vi "CANsub_WS_Close.vi"(7 "cert path":path=path "/home/lvuser/cansub_root_cert.crt", 8 "error in (no error)":errorcluster, 9 "channel":u8=2, 10 "host":string, 11 "TLS Connection":refnum<k5>) -> (0 "error out":errorcluster, 3 "closed by device":bool)   [LabVIEW 2021, in "CANsub_Common.lvlib"]
doc: "Closes the CANsub WebSocket: sends close frame 1000, reads until the device closes TCP (max 2 s), closes TCP. If the device did not close it, frees the channel with DELETE /api/can/<ch>/ws (200 or 404 OK). Always runs, also with an error in; the original error comes first in error out."
uses:
  CANsub_Common.lvlib
  <vilib>/httpClient/LabVIEWHTTPClient.lvlib
  Typedefs/HTTP_Method.ctl
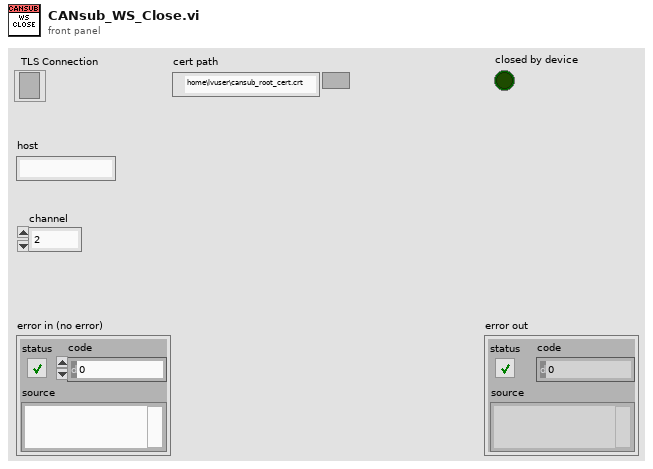
[diagram p1: front panel]
types:
  T1 = enum16{"Standard", "Buffered", "CRLF", "Immediate"}
  T2 = typedef "CANsub_Common.lvlib/HTTP_Method.ctl" = enum16{"GET", "PUT", "POST", "DELETE"}
  T3 = typedef "LabVIEWHTTPClient.lvlib/ClientHandle.ctl" = refnum<k1>
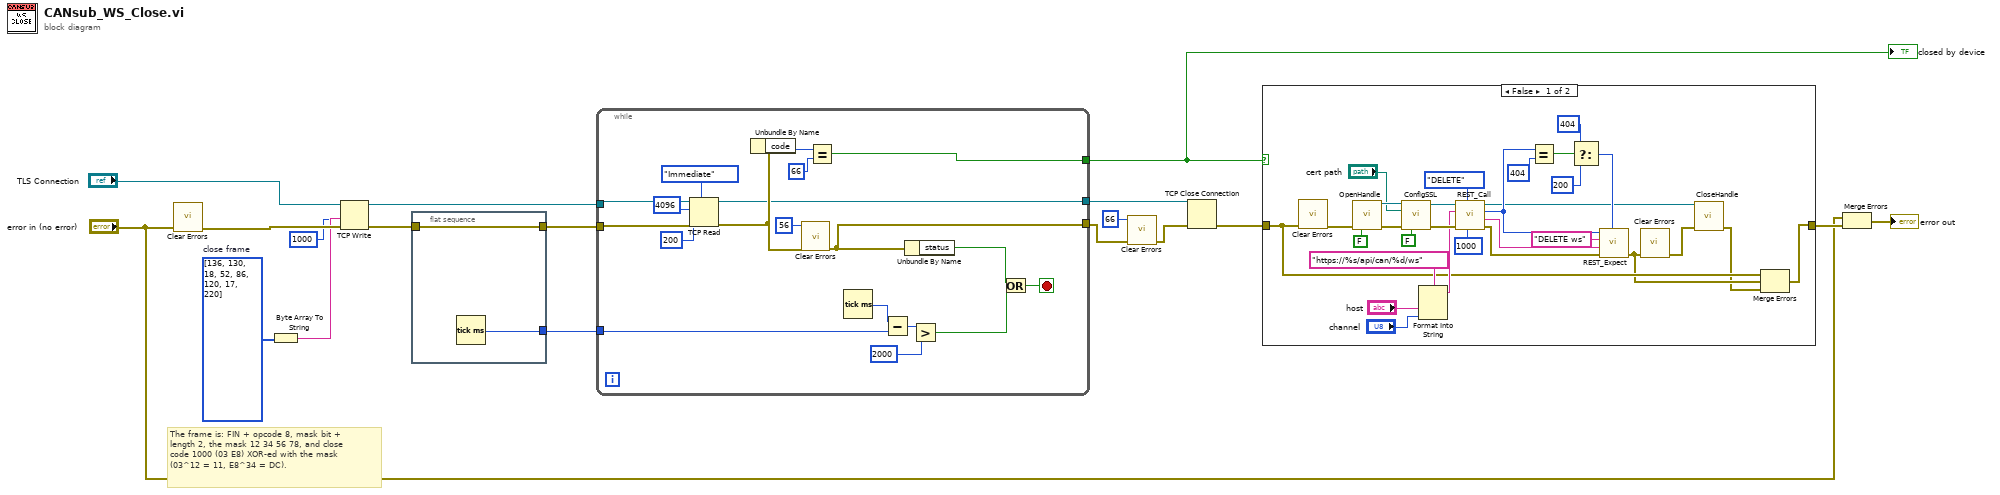
[diagram p0: block diagram]
diagram:
  w18 = u8[] [136, 130, 18, 52, 86, 120, 17, 220]  # close frame
  # "The frame is: FIN + opcode 8, mask bit + length 2, the mask 12 34 56 78, and close code 1000 (03 E8) XOR-ed with the mask (03^12 = 11, E8^34 = DC)."
  n1 = call <vilib>:"Clear Errors.vi"("error in (no error)"="error in (no error)") -> ("error out"=w17:errorcluster)  [unwired: 5 in, 1 out]
  n2 = Byte Array To String(unsigned byte array=w18) -> (string=w15:string)
  n3 = TCP Write(connection ID="TLS Connection", data in=w15, error in (no error)=w17, 9:1000 ("timeout ms (25000)")) -> (connection ID out=w7:refnum<k5>, error out=w13:errorcluster)  [unwired: 1 out]
  n4 = flat-sequence {
    tunnel: w13 -> [w20]
    tunnel: [w20] -> w11
    tunnel: [w19] -> w10
    frame #0 {
      n5 = Tick Count (ms)() -> (millisecond timer value=w19:u32)
    }
  }
  n6 = while {
    tunnel: w11 -> [w37]
    tunnel: w7 -> [w34]
    tunnel: w10 -> [w29]
    tunnel: [w23] -> w9
    tunnel: [w22] -> w2
    tunnel: [w21] -> w1
    stop <- w24 stop-if-true
    n7 = TCP Read(connection ID=w34, bytes to read=4096, error in (no error)=w37, 7:T1."Immediate" ("mode (standard)"), 9:200 ("timeout ms (25000)")) -> (connection ID out=w21:refnum<k5>, error out=w31:errorcluster)  [unwired: 1 out]
    n8 = Unbundle By Name(w31) -> ("code"=w33:i32)
    n9 = call <vilib>:"Clear Errors.vi"("error in (no error)"=w31, "specific error code to clear (0: all)"=56) -> ("error out"=w23:errorcluster)  [unwired: 4 in, 1 out]
    n10 = Equal?(x=w33, y=66) -> (x = y?=w22:bool)
    n11 = Tick Count (ms)() -> (millisecond timer value=w30:u32)
    n12 = Subtract(x=w30, y=w29) -> (x-y=w28:u32)
    n13 = Unbundle By Name(w23) -> ("status"=w26:bool)
    n14 = Greater?(x=w28, y=u32 2000) -> (0:w25:bool)
    n15 = Or(x=w26, y=w25) -> (x .or. y?=w24:bool)
  }
  "closed by device" <- w2
  n16 = call <vilib>:"Clear Errors.vi"("error in (no error)"=w9, "specific error code to clear (0: all)"=66) -> ("error out"=w8:errorcluster)  [unwired: 4 in, 1 out]
  n17 = TCP Close Connection(connection ID=w1, error in (no error)=w8) -> (error out=w6:errorcluster)  [unwired: 1 in, 1 out]
  n18 = case shown="False" w2 {
    tunnel: w6 -> [w44 w69]
    tunnel: [w41 w69] -> w5
    frame False {
      n19 = call <vilib>:"Clear Errors.vi"("error in (no error)"=w44) -> ("error out"=w68:errorcluster)  [unwired: 5 in, 1 out]
      n20 = call <vilib>:"OpenHandle.vi"("error in (no error)"=w68, "verify server(true)"=FALSE) -> ("client handle out"=w66:T3, "error out"=w65:errorcluster)  [unwired: 12 in]
      n21 = call <vilib>:"ConfigSSL.vi"("client handle"=w66, "CA certificate file"="cert path", "error in (no error)"=w65, "verify server (true)"=FALSE) -> ("client handle out"=w61:T3, "error out"=w62:errorcluster)  [unwired: 10 in]
      n22 = Format Into String(format string="https://%s/api/can/%d/ws", "host", "channel") -> (resulting string=w56:string)  [unwired: 2 in, 1 out]
      n23 = call "REST_Call.vi"("timeout ms (5000)"=1000, "method"=HTTP_Method."DELETE", "error in (no error)"=w62, "url"=w56, "client handle"=w61) -> ("error out"=w47:errorcluster, "response"=w48:string, "status"=w50:i32, "client handle out"=w45:T3)  [unwired: 3 in]
      n24 = Equal?(x=w50, y=404) -> (x = y?=w54:bool)
      n25 = Select(t=404 ("y"), s=w54, f=200 ("y")) -> (s? t:f=w51:i32)
      n26 = call "REST_Expect.vi"("expected"=w51, "error in (no error)"=w47, "response"=w48, "what"="DELETE ws", "status"=w50) -> ("error out"=w43:errorcluster)  [unwired: 5 in, 1 out]
      n27 = call <vilib>:"Clear Errors.vi"("error in (no error)"=w43) -> ("error out"=w46:errorcluster)  [unwired: 5 in, 1 out]
      n28 = call <vilib>:"CloseHandle.vi"("client handle"=w45, "error in (no error)"=w46) -> ("error out"=w42:errorcluster)  [unwired: 13 in]
      n29 = Merge Errors(w44, w43, w42) -> (w41:errorcluster)
    }
    frame True {
    }
  }
  n30 = Merge Errors("error in (no error)", w5) -> (→"error out":errorcluster)
